vi "RP1210 Send Message.vi"(6 "nBlockOnSend":i16, 7 "nNotifyStatusOnTx":i16, 8 "error in (no error)":errorcluster, 9 "nMessageSize":i16, 10 "fpchClientMessage":u8[](array[numeric])=array[4097 elements], 11 "nClientID":i16) -> (0 "error out":errorcluster, 3 "function return":i16)   [LabVIEW 2020, in "cansub_rp1210.lvlib"]
doc: "short __stdcall RP1210_SendMessage(short nClientID, unsigned char fpchClientMessage[], short nMessageSize,\n short nNotifyStatusOnTx, short nBlockOnSend);"
uses:
  cansub_rp1210.lvlib
  cansub_lv64.dll
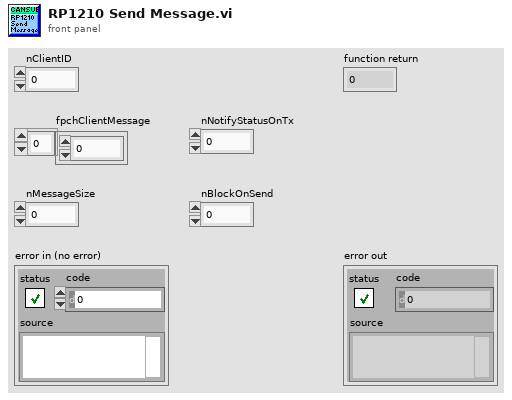
[diagram p1: front panel]
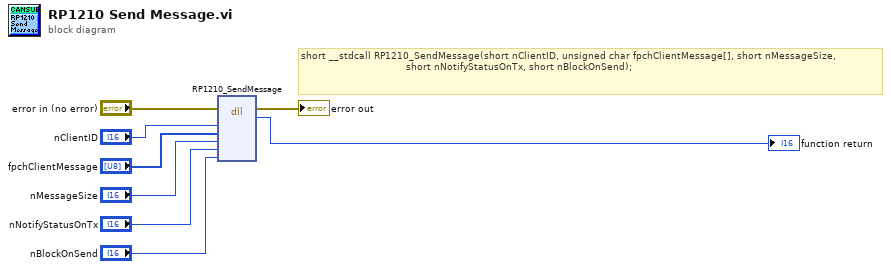
[diagram p0: block diagram]
diagram:
  # "short __stdcall RP1210_SendMessage(short nClientID, unsigned char fpchClientMessage[], short nMessageSize,\n                                   short nNotifyStatusOnTx, short nBlockOnSend);"
  n1 = dll-call lib="C:/cansub-lv/library/cansub_lv*.*" fn="RP1210_SendMessage"(error in="error in (no error)", "nClientID"="nClientID", "fpchClientMessage"="fpchClientMessage", "nMessageSize"="nMessageSize", "nNotifyStatusOnTx"="nNotifyStatusOnTx", "nBlockOnSend"="nBlockOnSend") -> (error out=→"error out":errorcluster, "return type"=→"function return":i16)  [unwired: 7 in, 1 out]
